vi "test Check If Custom Device is Enabled.vi"(8 "error in":errorcluster, 11 "TestCase in":refnum<class "Scripting.lvclass">) -> (0 "error out":errorcluster)   [LabVIEW 2020, in "Scripting.lvclass"]
uses:
  Scripting.lvclass
  Scripting.lvclass/Scripting.ctl
  Scripting/Ballard/Ballard ARINC 429 Scripting.lvlib
  <vilib>/addons/_JKI Toolkits/VI Tester/TestCase.llb/TestCase.lvclass
  C:/Program Files (x86)/National Instruments/LabVIEW 2020/vi.lib/addons/_JKI Toolkits/VI Tester/TestCase.llb/TestCase.lvclass
panel:
  out "TestCase out":refnum<class "Scripting.lvclass">
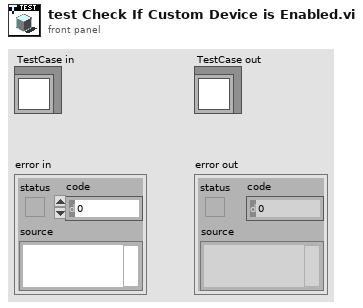
[diagram p1: front panel]
types:
  T1 = typedef "Custom Device API.lvlib/Custom Device Item Ref.ctl" = u64
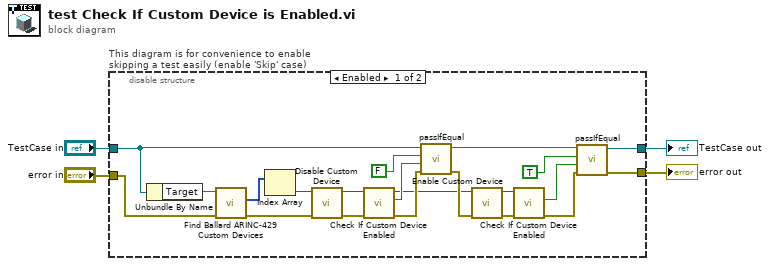
[diagram p0: block diagram]
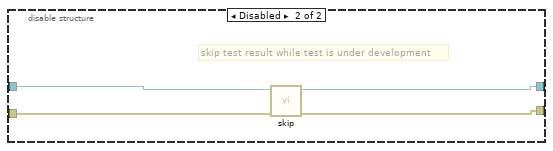
[diagram p2: hidden frame]
diagram:
  n1 = disable-structure "This diagram is for convenience to enable skipping a test easily (enable 'Skip' case)" shown="Enabled" {
    disable-tunnel: "TestCase in" -> [w19 w29]
    disable-tunnel: [w6 w27] -> w1
    disable-tunnel: [w7 w28] -> w3
    disable-tunnel: "error in" -> [w25 w26]
    frame Enabled {
      n2 = Unbundle By Name(w19) -> ("Target"=w20:refnum<k24>)
      n3 = call "Find Ballard ARINC-429 Custom Devices.vi"("error in"=w25, "target in"=w20) -> ("error out"=w21:errorcluster, "Ballard ARINC 429 custom devices"=w23:u64[])  [unwired: 7 in, 1 out]
      n4 = Index Array(array=w23) -> (element=w22:u64)  [unwired: 1 in]
      n5 = call "Disable Custom Device.vi"("error in (no error)"=w21, "Ballard ARINC 429 ref"=w22) -> ("error out"=w18:errorcluster, "Ballard ARINC 429 ref out"=w17:T1)  [unwired: 8 in]
      n6 = call "Check If Custom Device Enabled.vi"("error in (no error)"=w18, "Ballard ARINC 429 ref"=w17) -> ("error out"=w14:errorcluster, "Is Custom Device Enabled?"=w16:bool, "Ballard ARINC 429 ref"=w13:T1)  [unwired: 7 in]
      n7 = call-dynamic "passIfEqual.vi"("error in (no error)"=w14, "y"=w16, "x"=FALSE, "TestCase in"=w19) -> ("error out"=w24:errorcluster, "TestCase out"=w5:refnum<class "Scripting.lvclass">)  [unwired: 6 in]
      n8 = call "Enable Custom Device.vi"("error in (no error)"=w24, "Ballard ARINC 429 ref"=w13) -> ("error out"=w11:errorcluster, "Ballard ARINC 429 ref out"=w10:T1)  [unwired: 8 in]
      n9 = call "Check If Custom Device Enabled.vi"("error in (no error)"=w11, "Ballard ARINC 429 ref"=w10) -> ("error out"=w9:errorcluster, "Is Custom Device Enabled?"=w8:bool)  [unwired: 7 in, 1 out]
      n10 = call-dynamic "passIfEqual.vi"("error in (no error)"=w9, "y"=w8, "x"=TRUE, "TestCase in"=w5) -> ("error out"=w7:errorcluster, "TestCase out"=w6:refnum<class "Scripting.lvclass">)  [unwired: 6 in]
    }
    frame Disabled {
      # "skip test result while test is under development"
      n11 = call <vilib>:"skip.vi"("error in (no error)"=w26, "TestCase in"=w29) -> ("error out"=w28:errorcluster, "TestCase out"=w27:refnum<class "Scripting.lvclass">)  [unwired: 8 in]
    }
  }
  "error out" <- w3
  "TestCase out" <- w1
